vi "Swerve IMU Orientation Correction.vi"(9 "Setpoint":dbl format="%.2f", 10 "Robot Velocities In":T2) -> (2 "Robot Velocities Out":T2)   [LabVIEW 2025]
uses:
  Type Definitions/Data/Robot Velocities.ctl
  Robot Code/Framework/Robot Global Data.vi
panel:
  in  "output range":cluster{"high":dbl, "low":dbl}={"high"=100.0, "low"=-100.0} {"low" format="%.2f"; "high" format="%.2f"}
  in  "advanced":cluster{"alpha":dbl, "i-zone":dbl}={"alpha"=nan, "i-zone"=nan} {"i-zone" format="%.2f"; "alpha" format="%.2f"}
  in  "PID gains":T1={"proportional gain (Kp)"=10.0, "integral time (Ki)"=0.0, "derivative time (Kd)"=0.0} {"derivative time (Kd)" format="%.3f"; "integral time (Ki)" format="%.3f"; "proportional gain (Kp)" format="%.3f"}
  out "Err/Out Chart":cluster{dbl, dbl}(graph)
  out "SP/PV Chart":cluster{"setpoint":dbl, "process variable":dbl}(graph)
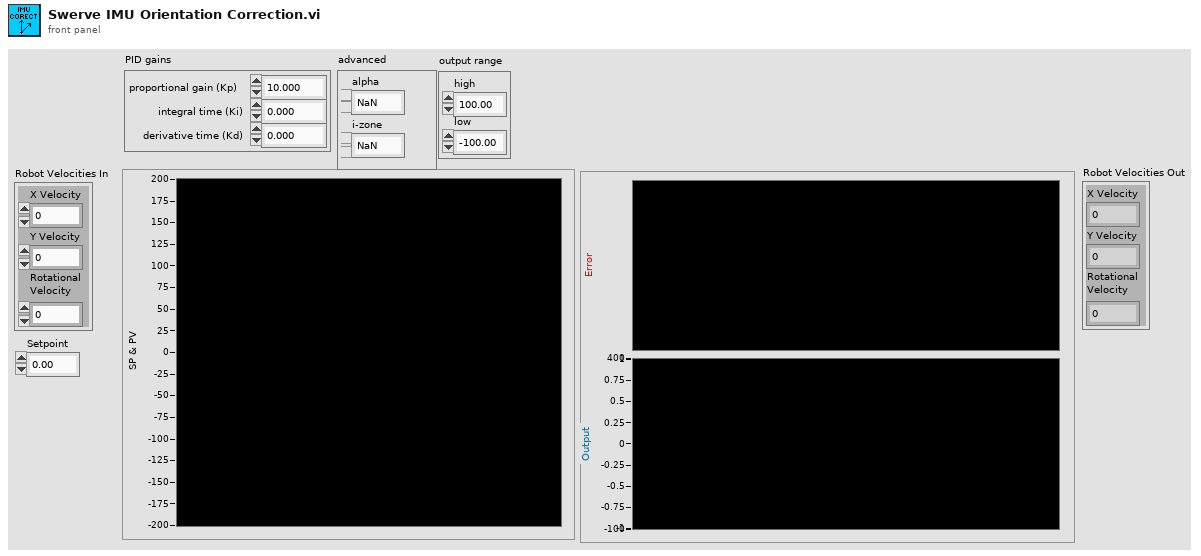
[diagram p1: front panel]
types:
  T1 = cluster{"proportional gain (Kp)":dbl, "integral time (Ki)":dbl, "derivative time (Kd)":dbl}
  T2 = typedef "Robot Velocities.ctl" = cluster{"X Velocity":dbl, "Y Velocity":dbl, "Rotational \nVelocity":dbl}
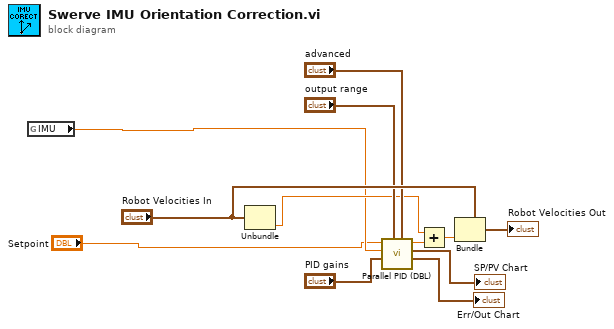
[diagram p0: block diagram]
diagram:
  n1 = global read "Robot Global Data.vi" "IMU"() -> (w2:dbl)
  n2 = Unbundle("Robot Velocities In") -> ("Rotational \nVelocity"=w4:dbl)  [unwired: 2 out]
  n3 = call <vilib>:"Parallel PID (DBL).vi"("advanced"="advanced", "output range"="output range", "PID gains"="PID gains", "process variable"=w2, "setpoint"="Setpoint") -> ("Err/Out Chart"=→"Err/Out Chart":cluster{dbl, dbl}, "SP/PV Chart"=→"SP/PV Chart":cluster{"setpoint":dbl, "process variable":dbl}, "output"=w5:dbl)  [unwired: 3 in, 1 out]
  n4 = Add(x=w4, y=w5) -> (x+y=w3:dbl)
  n5 = Bundle(cluster="Robot Velocities In", "Rotational \nVelocity"=w3) -> (→"Robot Velocities Out":T2)  [unwired: 2 in]
